vi "Tester - Is Element of Array.vi"() -> ()   [LabVIEW 2026, in "RSysUtils Array.lvlib"]
uses:
  RSysUtils Array.lvlib
  aabb578f-3a4f-4ec3-bf98-a8d83782f2fd.vi
  697f1e86-59ec-4e51-8f74-bb25258f2322.vi
  28c153bf-1dc1-4886-872d-0c7870bf2aaa.vi
  c32ec777-4d2a-4eab-af10-3d6aa8ee7525.vi
  e5a9c219-9d3c-4616-8c67-4212d7a67af3.vi
  ceb53368-45bc-49fb-af8b-05eb261a5257.vi
  75871626-3a6b-4915-a61f-05aedef905c5.vi
  2dc8f040-e328-4985-bba8-e31b96edccb7.vi
  d89310a1-3c34-450f-a9ef-b42a06342e9f.vi
  e6eb9be7-b027-48e0-ac8a-33517764eed0.vi
  c7daced9-db29-4f3e-949c-cfac833bea71.vi
  54c3fdeb-63da-4b96-a338-7af1d3c00d34.vi
  2e3c7274-ac8b-46da-bd7a-450313d87e0b.vi
  fc533ba3-13bb-409c-a81d-7436cfaae9a6.vi
  38027dd7-36cb-4a5a-a04b-e49a6caf8740.vi
  b28735d7-8d3d-430d-b74e-4f591f2f1183.vi
  905774d2-fe94-444e-9f16-8cf105834f6f.vi
  a603ebd2-6177-40a9-b1b1-45e868ad865f.vi
  eb546d27-330d-41c8-b84b-22c12632d17c.vi
  c9a44398-f4dc-4259-ab8a-7456e42347e3.vi
panel:
  out "Found? 20":bool
  out "Found? 19":bool
  out "Found? 18":bool
  out "Found? 17":bool
  out "Found? 16":bool
  out "3D Array":i32[][][](array[numeric])
  out "Found? 15":bool
  out "Found? 14":bool
  out "Found? 13":bool
  out "Found? 12":bool
  out "Found? 11":bool
  out "Found? 10":bool
  out "Found? 9":bool
  out "Found? 8":bool
  out "Found? 7":bool
  out "Found? 6":bool
  out "Found? 5":bool
  out "Found? 4":bool
  out "Found? 3":bool
  out "Found? 2":bool
  out "Found? 1":bool
  # "Tester - Is Element of Array"
  # "1D Array input"
  # "2D Array input"
  # "3D Array input"
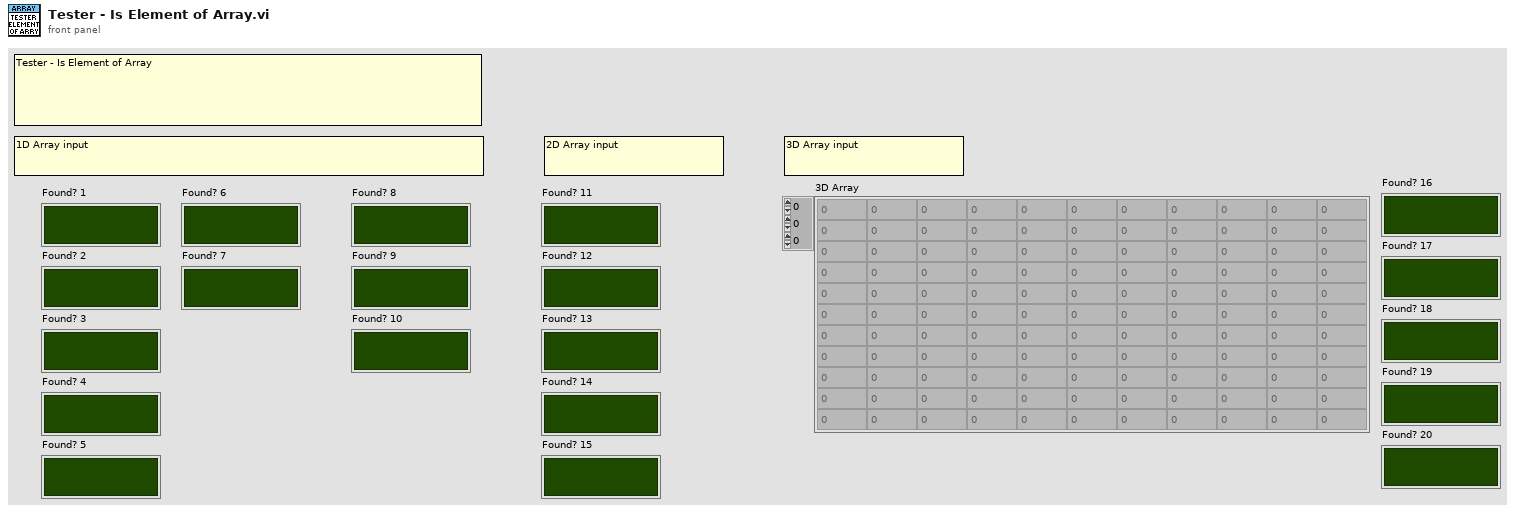
[diagram p1: front panel]
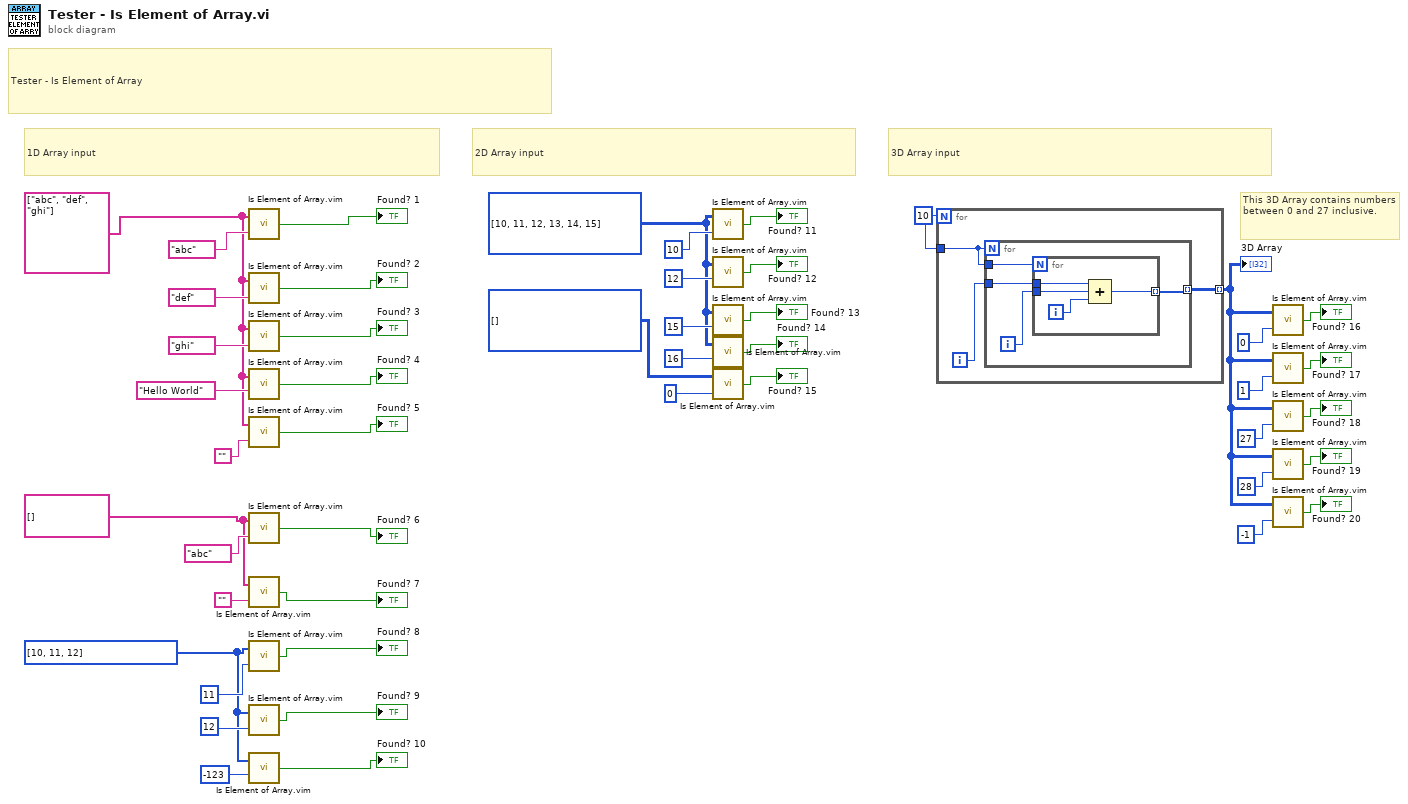
[diagram p0: block diagram]
diagram:
  w12 = 10
  w16 = i32[][] [[10, 11, 12], [13, 14, 15]]
  w27 = i32[] [10, 11, 12]
  w34 = string[] []
  w39 = string[] ["abc", "def", "ghi"]
  # "This 3D Array contains numbers between 0 and 27 inclusive."
  # "3D Array input"
  # "2D Array input"
  # "1D Array input"
  # "Tester - Is Element of Array"
  n1 = call "Is Element of Array.vim"("Element"="abc", "Array"=w39) -> ("Found?"=→"Found? 1":bool)
  n2 = call "Is Element of Array.vim"("Element"="def", "Array"=w39) -> ("Found?"=→"Found? 2":bool)
  n3 = call "Is Element of Array.vim"("Element"="ghi", "Array"=w39) -> ("Found?"=→"Found? 3":bool)
  n4 = call "Is Element of Array.vim"("Element"="Hello World", "Array"=w39) -> ("Found?"=→"Found? 4":bool)
  n5 = call "Is Element of Array.vim"("Element"="", "Array"=w39) -> ("Found?"=→"Found? 5":bool)
  n6 = call "Is Element of Array.vim"("Element"="abc", "Array"=w34) -> ("Found?"=→"Found? 6":bool)
  n7 = call "Is Element of Array.vim"("Element"="", "Array"=w34) -> ("Found?"=→"Found? 7":bool)
  n8 = call "Is Element of Array.vim"("Element"=11, "Array"=w27) -> ("Found?"=→"Found? 8":bool)
  n9 = call "Is Element of Array.vim"("Element"=12, "Array"=w27) -> ("Found?"=→"Found? 9":bool)
  n10 = call "Is Element of Array.vim"("Element"=-123, "Array"=w27) -> ("Found?"=→"Found? 10":bool)
  n11 = call "Is Element of Array.vim"("Element"=10, "Array"=w16) -> ("Found?"=→"Found? 11":bool)
  n12 = call "Is Element of Array.vim"("Element"=12, "Array"=w16) -> ("Found?"=→"Found? 12":bool)
  n13 = call "Is Element of Array.vim"("Element"=15, "Array"=w16) -> ("Found?"=→"Found? 13":bool)
  n14 = call "Is Element of Array.vim"("Element"=16, "Array"=w16) -> ("Found?"=→"Found? 14":bool)
  n15 = call "Is Element of Array.vim"("Element"=0, "Array"=i32[][] []) -> ("Found?"=→"Found? 15":bool)
  n16 = for {
    N: w12 -> [_]
    tunnel: w12 -> [w50]
    tunnel: [w48] -> w1 mode=indexing
    i -> [w49]
    n17 = for {
      N: w50 -> [_]
      tunnel: w50 -> [w54]
      tunnel: w49 -> [w53]
      tunnel: [w51] -> w48 mode=indexing
      i -> [w52]
      n18 = for {
        N: w54 -> [_]
        tunnel: w53 -> [w57]
        tunnel: w52 -> [w56]
        tunnel: [w55] -> w51 mode=indexing
        i -> [w58]
        n19 = Compound Arithmetic op=ADD(w57, w56, w58) -> (w55:i32)
      }
    }
  }
  "3D Array" <- w1
  n20 = call "Is Element of Array.vim"("Element"=0, "Array"=w1) -> ("Found?"=→"Found? 16":bool)
  n21 = call "Is Element of Array.vim"("Element"=1, "Array"=w1) -> ("Found?"=→"Found? 17":bool)
  n22 = call "Is Element of Array.vim"("Element"=27, "Array"=w1) -> ("Found?"=→"Found? 18":bool)
  n23 = call "Is Element of Array.vim"("Element"=28, "Array"=w1) -> ("Found?"=→"Found? 19":bool)
  n24 = call "Is Element of Array.vim"("Element"=-1, "Array"=w1) -> ("Found?"=→"Found? 20":bool)
